vi "String to Match Pattern Case Insensitive.vi"(1 "Input String":string) -> (0 "String":string)   [LabVIEW 2019, in "Error Generation.lvlib"]
doc: "- - -\nCopyright (c) 2023, Merecs Engineering GmbH"
uses:
  Error Generation.lvlib
panel:
  # "Connector Pane"
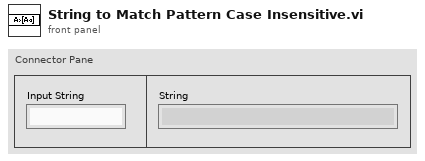
[diagram p1: front panel]
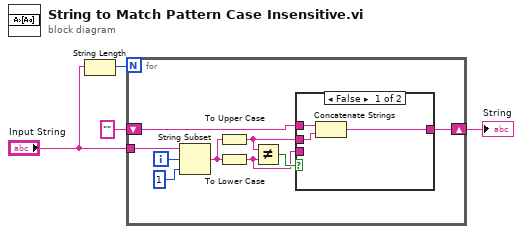
[diagram p0: block diagram]
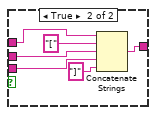
[diagram p2: hidden frame]
diagram:
  n1 = String Length(string="Input String") -> (length=w4:i32)
  n2 = for {
    N: w4 -> [_]
    tunnel: "Input String" -> [w12]
    shift-right: [w9] -> w1
    shift-left: "" -> [w8]
    i -> [w11]
    n3 = String Subset(string=w12, offset (0)=w11, length (rest)=1 ("length (rest)")) -> (substring=w10:string)
    n4 = To Upper Case(1:w10) -> (0:w6:string)
    n5 = To Lower Case(string=w10) -> (all lower case string=w5:string)
    n6 = Not Equal?(x=w6, y=w5) -> (x != y?=w7:bool)
    n7 = case shown="False" w7 {
      tunnel: w6 -> [w15 w22]
      tunnel: w5 -> [_ w21]
      tunnel: [w14 w18] -> w9
      tunnel: w8 -> [w16 w17]
      frame False {
        n8 = Concatenate Strings(w16, w15) -> (w14:string)
      }
      frame True {
        n9 = Concatenate Strings(w17, "[" ("string"), w22, w21, "]" ("string")) -> (w18:string)
      }
    }
  }
  "String" <- w1
